vi "G4BaseTemplate_Singleton_4x4x4_ReadAttribute.vi"(8 "Error In":errorcluster) -> (0 "Error Out":errorcluster)   [LabVIEW 2020]
uses:
  G4BaseTemplate_Singleton_4x4x4.lvclass
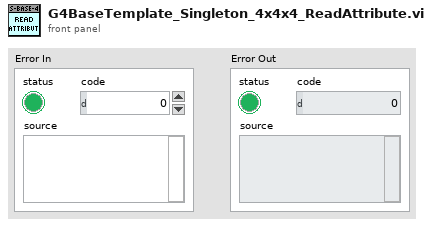
[diagram p1: front panel]
types:
  T1 = typedef "G4BaseTemplate_Singleton_4x4x4.lvclass/ObjectAttributes.ctl" = cluster{"Attribute1":dbl}
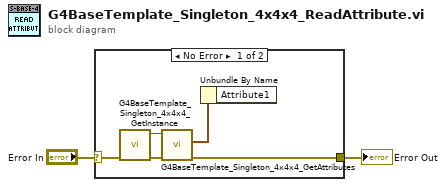
[diagram p0: block diagram]
diagram:
  n1 = case shown="No Error" "Error In" {
    selector: "Error In" -> [w4 w8]
    tunnel: [w6 w8] -> w1
    frame No Error {
      n2 = call "G4BaseTemplate_Singleton_4x4x4_GetInstance.vi"("Error In"=w4) -> ("Error Out"=w3:errorcluster, "reference out"=w5:refnum<class "G4BaseTemplate_Singleton_4x4x4.lvclass">)  [unwired: 6 in, 3 out]
      n3 = call "G4BaseTemplate_Singleton_4x4x4_GetAttributes.vi"("Error In"=w3, "reference in"=w5) -> ("Error Out"=w6:errorcluster, "Data"=w7:T1)  [unwired: 6 in, 2 out]
      n4 = Unbundle By Name(w7) -> ()  [unwired: 1 out]
    }
    frame Error {
    }
  }
  "Error Out" <- w1
